vi "Configure AI Timing.vi"(8 "error in (no error)":errorcluster, 11 "Task in":refnum<k21>) -> (0 "error out":errorcluster, 2 "AI Timing Settings":string, 3 "Task out":refnum<k21>)   [LabVIEW 2021, in "Load Frame.lvlib"]
doc: "Configure the timing settings for the AI task."
uses:
  Load Frame.lvlib
  <resource>/objmgr/daqmx.rc
  <vilib>/DAQmx/configure/timing.llb/DAQmx Timing (Sample Clock).vi
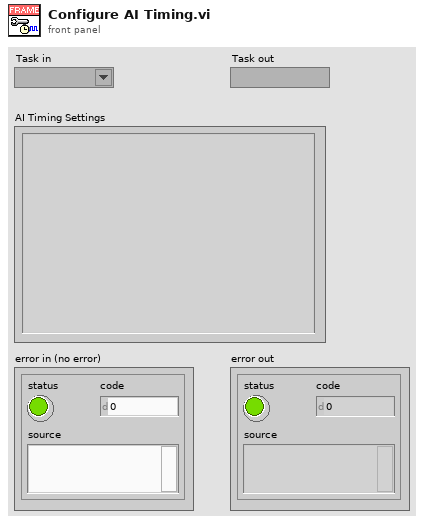
[diagram p1: front panel]
types:
  T1 = cluster{"SampClk.Rate":dbl, "SampClk.MaxRate":dbl}
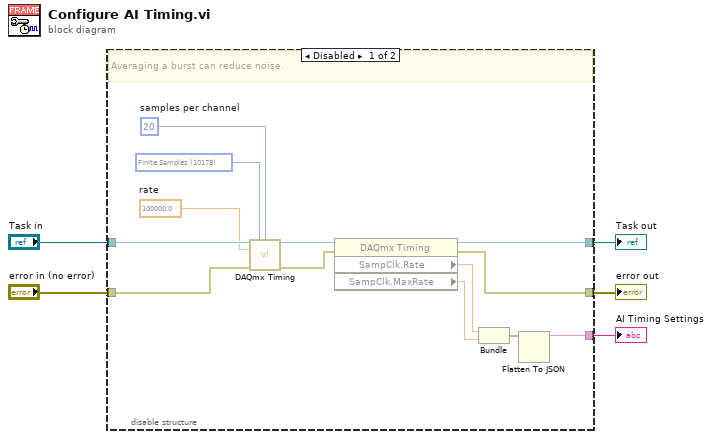
[diagram p0: block diagram]
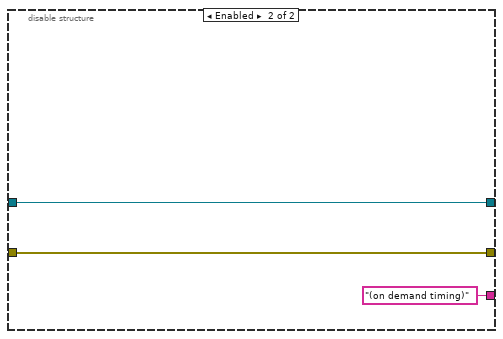
[diagram p2: hidden frame]
diagram:
  n1 = disable-structure shown="Disabled" {
    disable-tunnel: [w18 w21] -> w5
    disable-tunnel: [w16 w20] -> w4
    disable-tunnel: "error in (no error)" -> [w14 w20]
    disable-tunnel: "Task in" -> [w13 w21]
    disable-tunnel: [w7 "(on demand timing)" ("AI Timing Settings")] -> w1
    frame Disabled {
      w12 = 100000.0  # rate
      w11 = 20  # samples per channel
      w10 = 10178 items=["Finite Samples"=10178, "Continuous Samples"=10123, "Hardware Timed Single Point"=12522] ("sample mode")
      # "Averaging a burst can reduce noise."
      n2 = call-poly <vilib>:"DAQmx Timing.vi"("task/channels in"=w13, "sample mode"=w10, "samples per channel"=w11, "rate"=w12, "error in"=w14) -> ("task out"=w17:refnum<k21>, "error out"=w15:errorcluster)  [unwired: 9 in]
      n3 = property class="DAQmx Timing"(reference=w17, error in=w15) -> (reference out=w18:refnum<k21>, error out=w16:errorcluster, "SampClk.Rate"=w9:dbl, "SampClk.MaxRate"=w8:dbl)
      n4 = Bundle("SampClk.Rate"=w9, "SampClk.MaxRate"=w8) -> (w6:T1)  [unwired: 1 in]
      n5 = Flatten To JSON(anything=w6) -> (JSON string=w7:string)  [unwired: 2 in, 1 out]
    }
    frame Enabled {
    }
  }
  "Task out" <- w5
  "error out" <- w4
  "AI Timing Settings" <- w1
